vi "VIH HelpGen - FILE - Copy or Update File.vi"(8 "error in":errorcluster, 10 "Target Path":path, 11 "Source Path":path) -> (0 "error out":errorcluster, 3 "Target Path out":path)   [LabVIEW 2014]
doc: "::: VI Helpeks :::\nCopyright (c) 2000-2026 Konstantin Shifershteyn. All rights reserved."
panel:
  # "VI Helpeks\nCopyright (c) 2012-2026 Konstantin Shifershteyn"
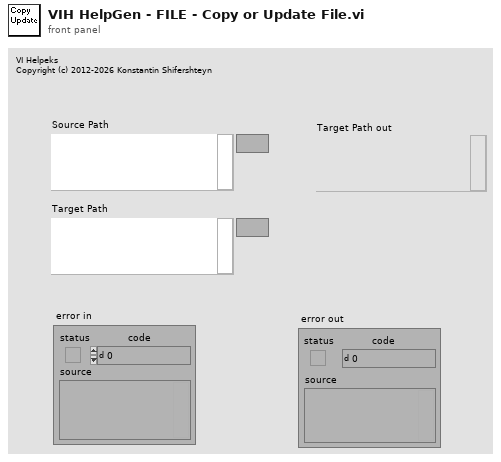
[diagram p1: front panel]
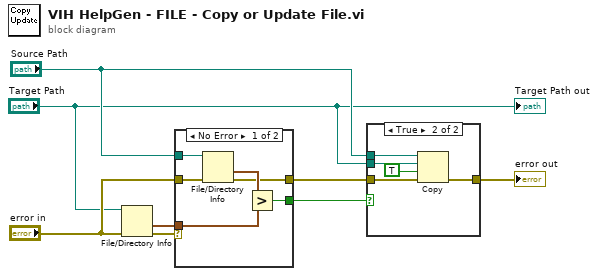
[diagram p0: block diagram]
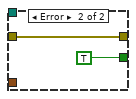
[diagram p3: hidden frame]
diagram:
  n1 = File/Directory Info(path="Target Path", error in="error in") -> (last mod=w7:timestamp, error out=w8:errorcluster)  [unwired: 5 out]
  n2 = case shown="No Error" w8 {
    tunnel: "Source Path" -> [w14 _]
    tunnel: w7 -> [w12 _]
    tunnel: [w11 TRUE] -> w4
    tunnel: [w10 w15] -> w6
    tunnel: "error in" -> [w9 w15]
    frame No Error {
      n3 = File/Directory Info(path=w14, error in=w9) -> (last mod=w13:timestamp, error out=w10:errorcluster)  [unwired: 5 out]
      n4 = Greater?(x=w13, y=w12) -> (0:w11:bool)
    }
    frame Error {
    }
  }
  n5 = case shown="True" w4 {
    tunnel: w6 -> [w17 w22]
    tunnel: [w17 w21] -> w2
    tunnel: "Source Path" -> [_ w20]
    tunnel: "Target Path" -> [_ w19]
    frame False {
    }
    frame True {
      n6 = Copy(8:w22, 9:TRUE, 10:w19, 11:w20) -> (0:w21:errorcluster)  [unwired: 1 in, 2 out]
    }
  }
  "error out" <- w2
  "Target Path out" <- "Target Path"
